vi "Flame step motor.vi"(2 "燃烧室控制电机地址":refnum<visa-resource-name>="COM2", 4 "X/Y":bool, 5 "Distance (mm)":sgl=10.0 format="%.2f") -> (1 "Position":sgl=151.00313 format="%.2f")   [LabVIEW 2020]
uses:
  <vilib>/Instr/_visa.llb/VISA Configure Serial Port (Instr).vi
panel:
  out "error out 2":errorcluster={"status"=FALSE, "code"=1073676294, "source"="VISA Read in Flame step motor.vi"}
  out "Position_String":string="?X\rX+96642\n"
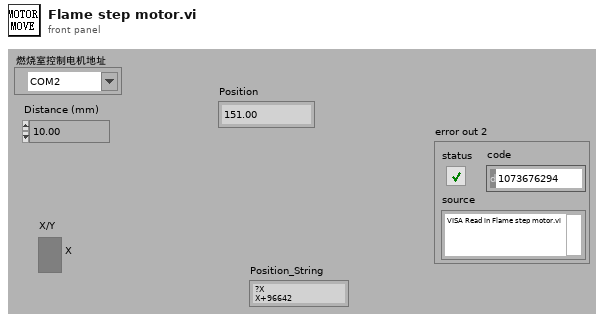
[diagram p1: front panel]
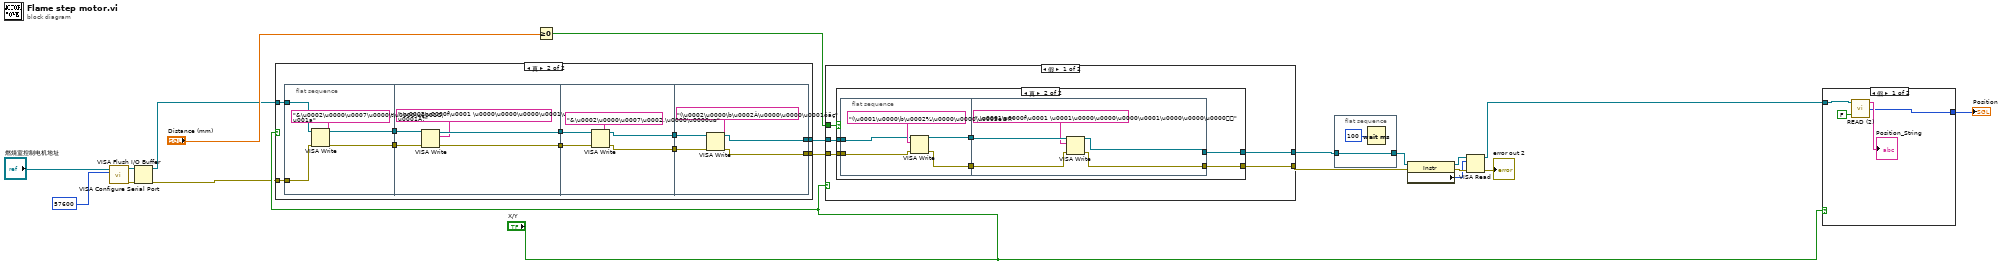
[diagram p0: block diagram]
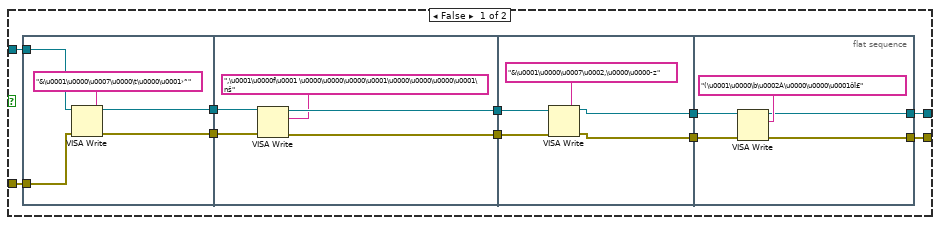
[diagram p2: hidden frame]
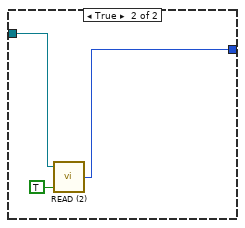
[diagram p3: hidden frame]
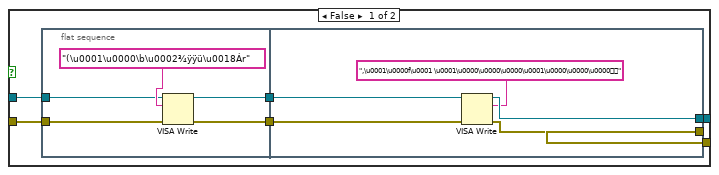
[diagram p4: hidden frame]
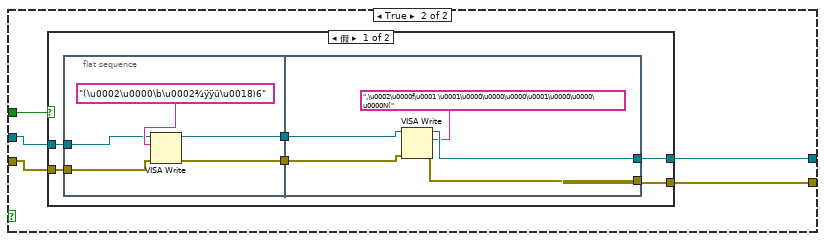
[diagram p5: hidden frame]
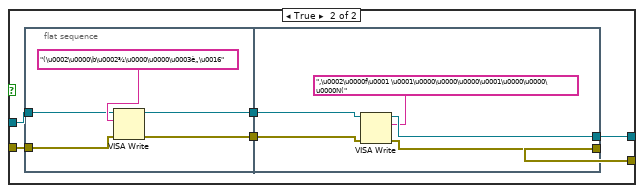
[diagram p6: hidden frame]
diagram:
  n1 = call-poly "VISA Configure Serial Port"("VISA resource name"="燃烧室控制电机地址", "baud rate (9600)"=u32 57600) -> ("VISA resource name out"=w13:refnum<visa-resource-name>, "error out"=w3:errorcluster)  [unwired: 12 in]
  n2 = VISA Flush I/O Buffer(VISA resource name=w13, error in (no error)=w3) -> (VISA resource name out=w1:refnum<visa-resource-name>, error out=w7:errorcluster)  [unwired: 1 in]
  n3 = case shown="真" "X/Y" {
    tunnel: w1 -> [w30 w60]
    tunnel: w7 -> [w29 w59]
    tunnel: [w22 w52] -> w5
    tunnel: [w21 w51] -> w4
    frame False {
      n4 = flat-sequence {
        tunnel: w30 -> [w35]
        tunnel: w29 -> [w34]
        tunnel: [w33] -> w28
        tunnel: [w32] -> w25
        tunnel: w28 -> [w40]
        tunnel: [w39] -> w27
        tunnel: w25 -> [w38]
        tunnel: [w37] -> w24
        tunnel: w27 -> [w45]
        tunnel: [w44] -> w26
        tunnel: w24 -> [w43]
        tunnel: [w42] -> w23
        tunnel: w26 -> [w50]
        tunnel: w23 -> [w49]
        tunnel: [w47] -> w22
        tunnel: [w46] -> w21
        frame #0 {
          n5 = VISA Write(VISA resource name=w35, write buffer="&\u0001\u0000\u0007\u0000\t\u0000\u0001›˜" ("写入缓冲区"), error in (no error)=w34) -> (VISA resource name out=w33:refnum<visa-resource-name>, error out=w32:errorcluster)  [unwired: 1 out]
        }
        frame #1 {
          n6 = VISA Write(VISA resource name=w40, write buffer=",\u0001\u0000f\u0001 \u0000\u0000\u0000\u0001\u0000\u0000\u0000\u0001\nš" ("写入缓冲区"), error in (no error)=w38) -> (VISA resource name out=w39:refnum<visa-resource-name>, error out=w37:errorcluster)  [unwired: 1 out]
        }
        frame #2 {
          n7 = VISA Write(VISA resource name=w45, write buffer="&\u0001\u0000\u0007\u0002‚\u0000\u0000­z" ("写入缓冲区"), error in (no error)=w43) -> (VISA resource name out=w44:refnum<visa-resource-name>, error out=w42:errorcluster)  [unwired: 1 out]
        }
        frame #3 {
          n8 = VISA Write(VISA resource name=w50, write buffer="(\u0001\u0000\b\u0002À\u0000\u0000\u0001ôÎ£" ("写入缓冲区"), error in (no error)=w49) -> (VISA resource name out=w47:refnum<visa-resource-name>, error out=w46:errorcluster)  [unwired: 1 out]
        }
      }
    }
    frame True {
      n9 = flat-sequence {
        tunnel: w60 -> [w65]
        tunnel: w59 -> [w64]
        tunnel: [w63] -> w58
        tunnel: [w62] -> w57
        tunnel: w58 -> [w70]
        tunnel: w57 -> [w69]
        tunnel: [w68] -> w56
        tunnel: [w67] -> w55
        tunnel: w56 -> [w75]
        tunnel: w55 -> [w74]
        tunnel: [w73] -> w54
        tunnel: [w72] -> w53
        tunnel: w54 -> [w80]
        tunnel: w53 -> [w79]
        tunnel: [w78] -> w52
        tunnel: [w77] -> w51
        frame #0 {
          n10 = VISA Write(VISA resource name=w65, write buffer="&\u0002\u0000\u0007\u0000\t\u0000\u0001C\u001a" ("写入缓冲区"), error in (no error)=w64) -> (VISA resource name out=w63:refnum<visa-resource-name>, error out=w62:errorcluster)  [unwired: 1 out]
        }
        frame #1 {
          n11 = VISA Write(VISA resource name=w70, write buffer=",\u0002\u0000f\u0001 \u0000\u0000\u0000\u0001\u0000\u0000\u0000\u0001Å?" ("写入缓冲区"), error in (no error)=w69) -> (VISA resource name out=w68:refnum<visa-resource-name>, error out=w67:errorcluster)  [unwired: 1 out]
        }
        frame #2 {
          n12 = VISA Write(VISA resource name=w75, write buffer="&\u0002\u0000\u0007\u0002‚\u0000\u0000uø" ("写入缓冲区"), error in (no error)=w74) -> (VISA resource name out=w73:refnum<visa-resource-name>, error out=w72:errorcluster)  [unwired: 1 out]
        }
        frame #3 {
          n13 = VISA Write(VISA resource name=w80, write buffer="(\u0002\u0000\b\u0002À\u0000\u0000\u0001ôãç" ("写入缓冲区"), error in (no error)=w79) -> (VISA resource name out=w78:refnum<visa-resource-name>, error out=w77:errorcluster)  [unwired: 1 out]
        }
      }
    }
  }
  n14 = Greater Or Equal To 0?(x="Distance (mm)") -> (x >= 0?=w12:bool)
  n15 = case shown="假" "X/Y" {
    tunnel: w12 -> [w85 w122]
    tunnel: [w84 w121] -> w18
    tunnel: [w83 w120] -> w14
    tunnel: w5 -> [w82 w119]
    tunnel: w4 -> [w81 w118]
    frame False {
      n16 = case shown="真" w85 {
        tunnel: [w87 w105] -> w83
        tunnel: [w86 w104] -> w84
        tunnel: w82 -> [w89 w103]
        tunnel: w81 -> [w88 w102]
        frame False {
          n17 = flat-sequence {
            tunnel: [w96] -> w91
            tunnel: [w95] -> w90
            tunnel: w89 -> [w93]
            tunnel: w88 -> [w92]
            tunnel: w91 -> [w100]
            tunnel: w90 -> [w101]
            tunnel: [w99] -> w87
            tunnel: [w98] -> w86
            frame #0 {
              n18 = VISA Write(VISA resource name=w93, write buffer="(\u0001\u0000\b\u0002¾ÿÿü\u0018Ár" ("写入缓冲区"), error in (no error)=w92) -> (VISA resource name out=w95:refnum<visa-resource-name>, error out=w96:errorcluster)  [unwired: 1 out]
            }
            frame #1 {
              n19 = VISA Write(VISA resource name=w101, write buffer=",\u0001\u0000f\u0001 \u0001\u0000\u0000\u0000\u0001\u0000\u0000\u0000" ("写入缓冲区"), error in (no error)=w100) -> (VISA resource name out=w99:refnum<visa-resource-name>, error out=w98:errorcluster)  [unwired: 1 out]
            }
          }
        }
        frame True {
          n20 = flat-sequence {
            tunnel: [w112] -> w107
            tunnel: [w111] -> w106
            tunnel: w103 -> [w109]
            tunnel: w102 -> [w108]
            tunnel: w107 -> [w114]
            tunnel: w106 -> [w115]
            tunnel: [w117] -> w105
            tunnel: [w116] -> w104
            frame #0 {
              n21 = VISA Write(VISA resource name=w109, write buffer="(\u0001\u0000\b\u0002¾\u0000\u0000\u0003è©R" ("写入缓冲区"), error in (no error)=w108) -> (VISA resource name out=w111:refnum<visa-resource-name>, error out=w112:errorcluster)  [unwired: 1 out]
            }
            frame #1 {
              n22 = VISA Write(VISA resource name=w115, write buffer=",\u0001\u0000f\u0001 \u0001\u0000\u0000\u0000\u0001\u0000\u0000\u0000" ("写入缓冲区"), error in (no error)=w114) -> (VISA resource name out=w117:refnum<visa-resource-name>, error out=w116:errorcluster)  [unwired: 1 out]
            }
          }
        }
      }
    }
    frame True {
      n23 = case shown="假" w122 {
        tunnel: [w126 w142] -> w120
        tunnel: [w125 w141] -> w121
        tunnel: w119 -> [w124 w140]
        tunnel: w118 -> [w123 w139]
        frame False {
          n24 = flat-sequence {
            tunnel: [w133] -> w128
            tunnel: [w132] -> w127
            tunnel: w124 -> [w130]
            tunnel: w123 -> [w129]
            tunnel: w128 -> [w137]
            tunnel: w127 -> [w138]
            tunnel: [w136] -> w126
            tunnel: [w135] -> w125
            frame #0 {
              n25 = VISA Write(VISA resource name=w130, write buffer="(\u0002\u0000\b\u0002¾ÿÿü\u0018ì6" ("写入缓冲区"), error in (no error)=w129) -> (VISA resource name out=w132:refnum<visa-resource-name>, error out=w133:errorcluster)  [unwired: 1 out]
            }
            frame #1 {
              n26 = VISA Write(VISA resource name=w138, write buffer=",\u0002\u0000f\u0001 \u0001\u0000\u0000\u0000\u0001\u0000\u0000\u0000N(" ("写入缓冲区"), error in (no error)=w137) -> (VISA resource name out=w136:refnum<visa-resource-name>, error out=w135:errorcluster)  [unwired: 1 out]
            }
          }
        }
        frame True {
          n27 = flat-sequence {
            tunnel: [w149] -> w144
            tunnel: [w148] -> w143
            tunnel: w140 -> [w146]
            tunnel: w139 -> [w145]
            tunnel: w144 -> [w153]
            tunnel: w143 -> [w154]
            tunnel: [w152] -> w142
            tunnel: [w151] -> w141
            frame #0 {
              n28 = VISA Write(VISA resource name=w146, write buffer="(\u0002\u0000\b\u0002¾\u0000\u0000\u0003è„\u0016" ("写入缓冲区"), error in (no error)=w145) -> (VISA resource name out=w148:refnum<visa-resource-name>, error out=w149:errorcluster)  [unwired: 1 out]
            }
            frame #1 {
              n29 = VISA Write(VISA resource name=w154, write buffer=",\u0002\u0000f\u0001 \u0001\u0000\u0000\u0000\u0001\u0000\u0000\u0000N(" ("写入缓冲区"), error in (no error)=w153) -> (VISA resource name out=w152:refnum<visa-resource-name>, error out=w151:errorcluster)  [unwired: 1 out]
            }
          }
        }
      }
    }
  }
  n30 = flat-sequence {
    tunnel: w14 -> [w156]
    tunnel: [w156] -> w15
    frame #0 {
      n31 = Wait (ms)(milliseconds to wait=u32 100) -> ()  [unwired: 1 out]
    }
  }
  n32 = property class="Instr"(reference=w15, error in=w18) -> (reference out=w16:refnum<visa-resource-name>, error out=w19:errorcluster, "Serial Settings:Number of Bytes at Serial Port"=w17:u32)
  n33 = VISA Read(VISA resource name=w16, byte count=w17, error in (no error)=w19) -> (VISA resource name out=w2:refnum<visa-resource-name>, error out=→"error out 2":errorcluster)  [unwired: 2 out]
  n34 = case shown="假" "X/Y" {
    tunnel: [w158 w162] -> w9
    tunnel: w2 -> [w160 w163]
    frame False {
      n35 = call "READ (2).vi"("X/Y"=FALSE, "VISA resource name"=w160) -> ("电机位置"=w158:u32, "读取缓冲区"=→"Position_String":string)  [unwired: 1 in, 1 out]
    }
    frame True {
      n36 = call "READ (2).vi"("X/Y"=TRUE, "VISA resource name"=w163) -> ("电机位置"=w162:u32)  [unwired: 1 in, 2 out]
    }
  }
  "Position" <- w9
